vi "Disable Frame0 Enabled.vi"(8 "error in":errorcluster) -> (0 "error out":errorcluster, 1 "Result":i32)   [LabVIEW 2026]
doc: "Issue 129 repro: a Diagram Disable Structure whose frame 0 is enabled."
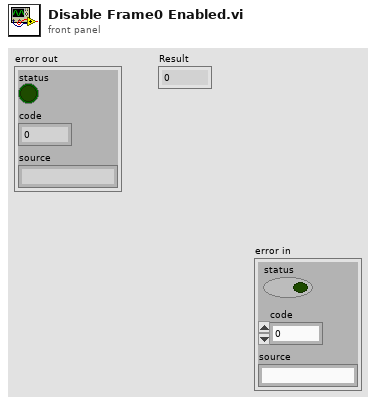
[diagram p1: front panel]
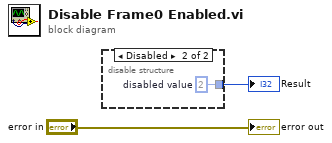
[diagram p0: block diagram]
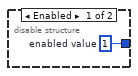
[diagram p2: hidden frame]
diagram:
  n1 = disable-structure shown="Disabled" {
    disable-tunnel: [w3 w4] -> w2
    frame Enabled {
      w3 = 1  # enabled value
    }
    frame Disabled {
      w4 = 2  # disabled value
    }
  }
  "Result" <- w2
  "error out" <- "error in"
